vi "Parse Results (single).vi"(6 "Datatype":T1, 8 "error in (no error)":errorcluster, 9 "Reference Channel":i32=1, 10 "AI Channel":i32=1, 11 "Results (Dictionary)":cluster{"key":string, "value":dbl}[](array[cluster])) -> (0 "error out":errorcluster, 1 "Name":string, 2 "Data":dbl, 3 "Results (Dictionary)":cluster{"key":string, "value":dbl}[](array[cluster]))   [LabVIEW 2019, in "Instrument.Lockin.lvlib" / "Instrument.Lockin.lvclass"]
doc: "This method will search the <b>Results Dictionary</b> for the data specified by <b>Datatype</b>, <b>AI Channel</b>, and <b>Ref Channel</b>.\n\n<b>Data</b> is either samples one point or takes the mean of the returned array values in the matched channel."
uses:
  Instrument.Lockin.lvclass
  Typedefs/Results Type--Enum.ctl
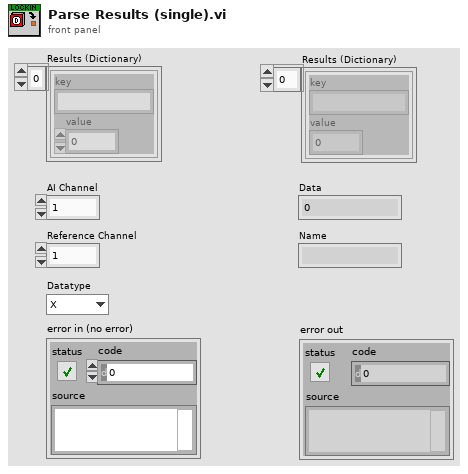
[diagram p1: front panel]
types:
  T1 = typedef "Instrument.Lockin.lvlib/Instrument.Lockin.lvclass/Results Type--Enum.ctl" = enum16{"X", "Y", "R", "Theta", "Mean"}
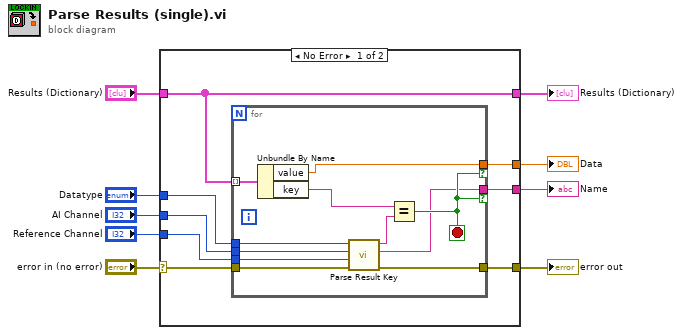
[diagram p0: block diagram]
diagram:
  n1 = case shown="No Error" "error in (no error)" {
    selector: "error in (no error)" -> [w13 w29]
    tunnel: "Datatype" -> [w16 _]
    tunnel: "Results (Dictionary)" -> [w17 w30]
    tunnel: [w14 _] -> w3
    tunnel: [w12 w29] -> w2
    tunnel: [w17 w30] -> w6
    tunnel: "Reference Channel" -> [w15 _]
    tunnel: "AI Channel" -> [w10 _]
    tunnel: [w11 _] -> w1
    frame No Error {
      n2 = for {
        tunnel: [w28] -> w11 if=w24
        tunnel: [w23] -> w14 if=w24
        tunnel: w17 -> [w27] mode=indexing
        tunnel: w10 -> [w19]
        tunnel: w15 -> [w18]
        tunnel: w16 -> [w26]
        tunnel: w13 -> [w22]
        tunnel: [w21] -> w12
        stop <- w24 stop-if-true
        n3 = Unbundle By Name(w27) -> ("value"=w28:dbl, "key"=w20:string)
        n4 = call "Parse Result Key.vi"("error in (no error)"=w22, "Ref Channel"=w18, "AI Channel"=w19, "Datatype"=w26) -> ("error out"=w21:errorcluster, "Label"=w23:string, "Key"=w25:string)  [unwired: 5 in]
        n5 = Equal?(x=w20, y=w25) -> (x = y?=w24:bool)
      }
    }
    frame Error {
    }
  }
  "Data" <- w1
  "Results (Dictionary)" <- w6
  "Name" <- w3
  "error out" <- w2
